vi "SA get TDF File List.vi"(8 "error in (no error)":errorcluster caption="에러 입력(에러 없음)", 11 "Instrument Manager 입력":refnum<class "Instrument Manager.lvclass">) -> (0 "error out":errorcluster caption="에러 출력", 3 "Instrument Manager 출력":refnum<class "Instrument Manager.lvclass">)   [LabVIEW 2023]
uses:
  Module/Spectrum Analyzer/Interface_Spectrum/Interface_Spectrum.lvclass
  Module/ANRITSU Call Box/Interface Class/Anritsu Call Box.lvclass
  Module/CE RF Switch Box/RF Filter Box/RF Filter Box.lvclass
  Module/Turn Table and Mast Control/Interface Class/Turn Table/Interface - Turn Table.lvclass
  Module/Turn Table and Mast Control/Interface Class/Mast/Interface - Mast.lvclass
  Module/FCC FR2 3D Controller Module/Interface_3D Controller/Interface_3D Controller.lvclass
  Instrument Manager.lvclass
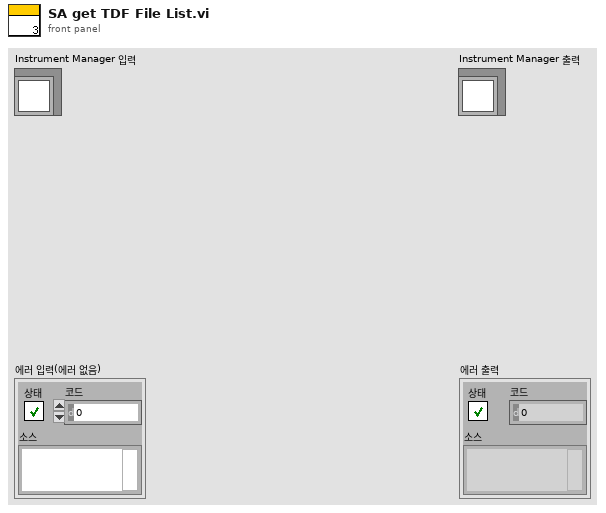
[diagram p1: front panel]
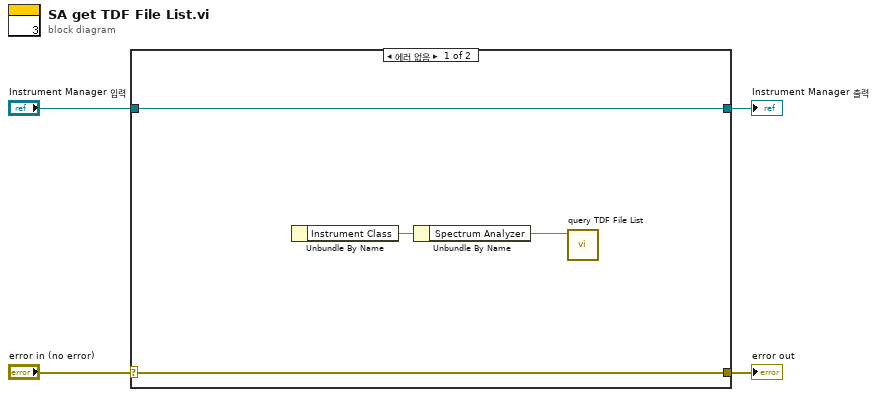
[diagram p0: block diagram]
diagram:
  n1 = case shown="에러 없음" "error in (no error)" {
    selector: "error in (no error)" -> [w7 w10]
    tunnel: [w7 w10] -> w3
    tunnel: [w8 w9] -> w1
    tunnel: "Instrument Manager 입력" -> [w8 w9]
    frame No Error {
      n2 = Unbundle By Name() -> ("Instrument Class"=w6)  [unwired: 1 in]
      n3 = Unbundle By Name(w6) -> ("Spectrum Analyzer"=w5)
      n4 = call-dynamic "query TDF File List.vi"("Interface_Spectrum 입력"=w5) -> ()  [unwired: 8 in, 3 out]
    }
    frame Error {
    }
  }
  "error out" <- w3
  "Instrument Manager 출력" <- w1
